vi "Beam Profiler.vi"(7 "Image Ref":T1) -> ()   [LabVIEW 2016]
uses:
  <vilib>/Utility/miscctls.llb/LVPointTypeDef.ctl
  <vilib>/vision/NI_Vision_Development_Module.lvlib
  <vilib>/vision/Image Controls.llb/IMAQ Image.ctl
panel:
  out "Y FWHM (px)":dbl=1.0
  out "X FWHM (px)":dbl=1.0
  out "Y FWHM (mm)":dbl=1.0
  out "X FWHM (mm)":dbl=1.0
  in  "Camera Pixel Size (µm)":dbl=1.0
  in  "Fitting":bool
  out "Fit":dbl[][](graph)
  out "Image":u16[][](graph)
  in  "Update Rate (ms)":i32=50
  in  "Binning (pixels)":i32=10 min=1 step=1
  in  "Done":bool
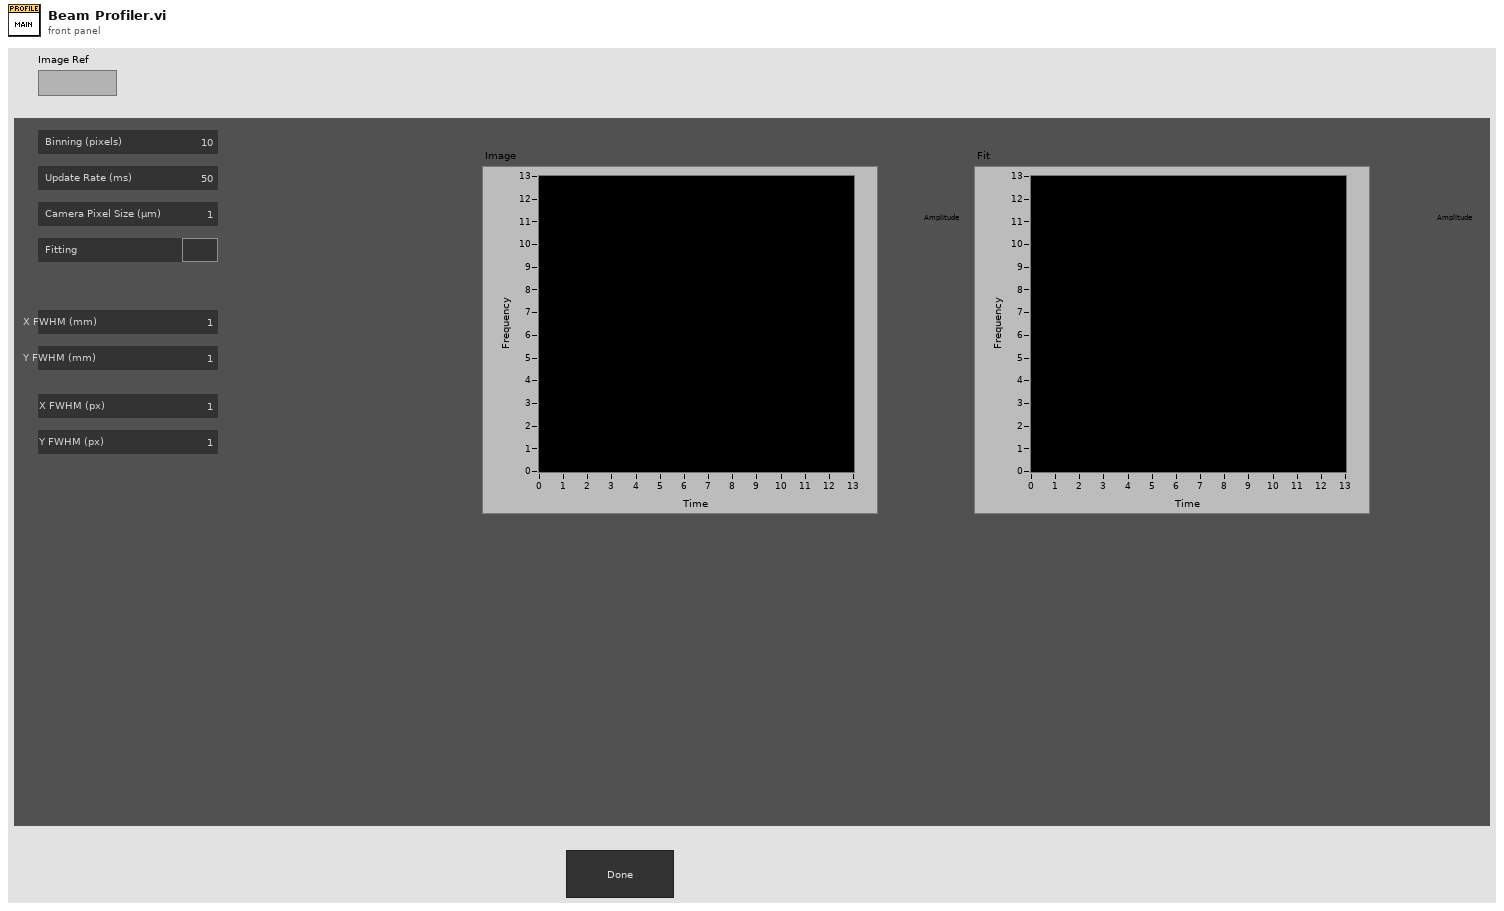
[diagram p1: front panel]
types:
  T1 = typedef "IMAQ Image.ctl" = refnum<image>
  T2 = typedef "Image Type" = u32
  T3 = enum16{"Always On", "Always Off", "Off While Running"}
  T4 = typedef "LVPointTypeDef.ctl" = cluster{"Horizontal":i16, "Vertical":i16}
  T5 = typedef "2D Gaussian - Best Fit Parameters.ctl" = cluster{"Amplitude":dbl, "X Position":dbl, "Y Position":dbl, "X Width":dbl, "Y Width":dbl, "Offset":dbl}
  T6 = typedef "LVRectTypeDef.ctl" = cluster{"Left":i16, "Top":i16, "Right":i16, "Bottom":i16}
  T7 = typedef "LVBoundsTypeDef.ctl" = cluster{"Width":u32, "Height":u32}
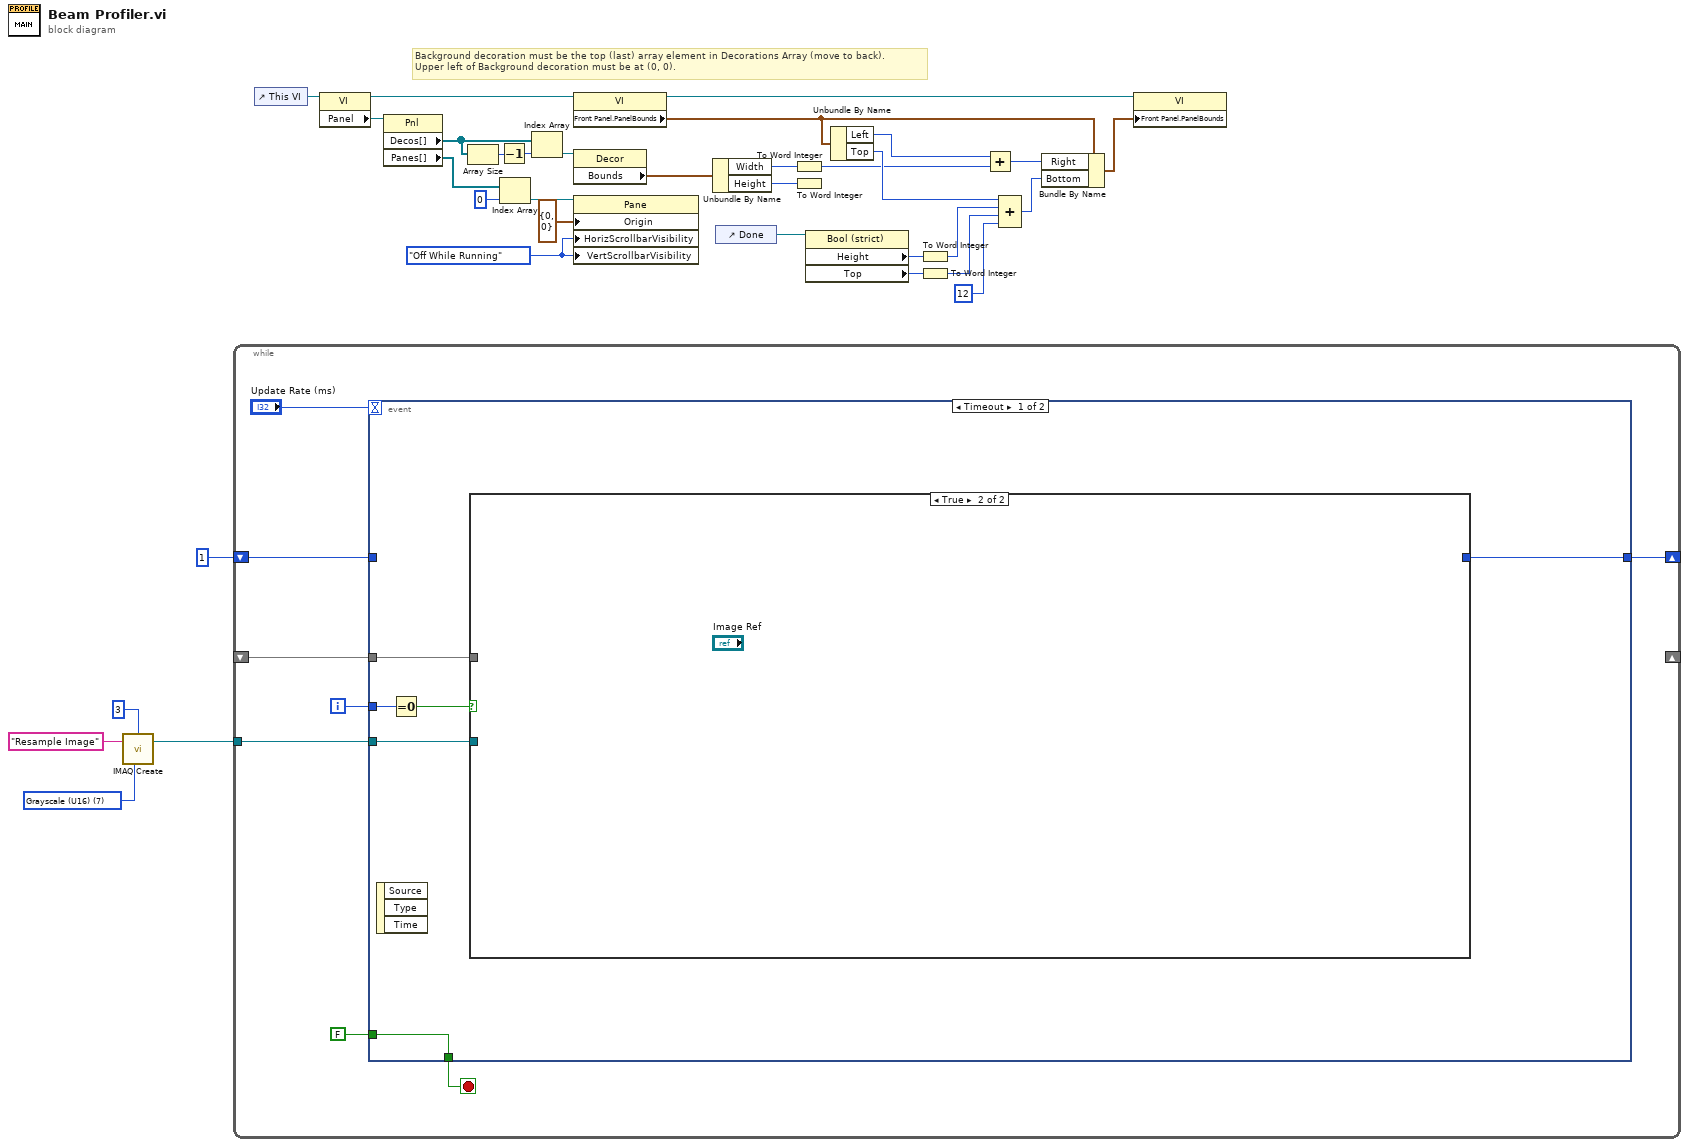
[diagram p0: block diagram]
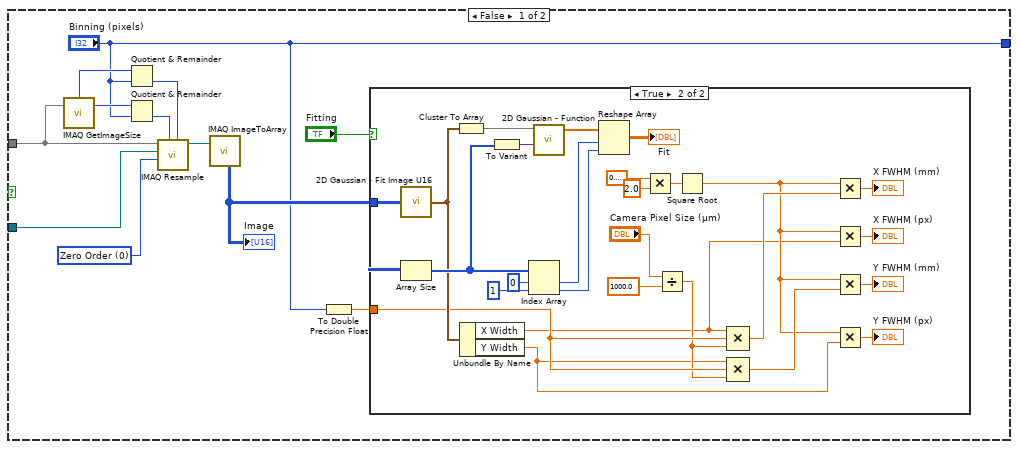
[diagram p2: hidden frame]
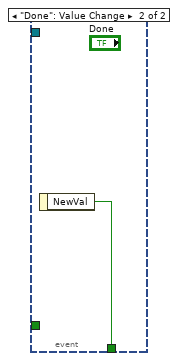
[diagram p4: hidden frame]
diagram:
  w5 = T2 7 items=["Grayscale (U8)", "Grayscale (I16)", "Grayscale (SGL)", "Complex (CSG)", "RGB (U32)", "HSL (U32)", "RGB (U64)", "Grayscale (U16)"] ("Image Type")
  w17 = T3."Off While Running" ("Vertical Scrollbar Visibility")
  # "Background decoration must be the top (last) array element in Decorations Array (move to back).\nUpper left of Background decoration must be at (0, 0)."
  n1 = call "IMAQ Create"("Border Size"=3, "Image Name"="Resample Image", "Image Type"=w5) -> ("New Image"=w2:T1)  [unwired: 2 in, 1 out]
  n2 = while {
    tunnel: w2 -> [w38]
    shift-right: _ -> [_]
    shift-left: _ -> [w39]
    shift-right: [w36] -> _
    shift-left: 1 ("Binning (pixels)") -> [w35]
    i -> [w37]
    stop <- w41 stop-if-true
    n3 = event shown="[0] Timeout" {
      selector: _ -> [_ _]
      dyn-events: _ -> [_ _]
      timeout: "Update Rate (ms)" -> [_ _]
      tunnel: [w48 w88] -> w41
      tunnel: FALSE -> [w48 _]
      tunnel: w39 -> [w46 _]
      tunnel: w38 -> [w47 _]
      tunnel: w37 -> [w45 _]
      tunnel: [w43 _] -> w36
      tunnel: w35 -> [_ _]
      event Timeout {
        n4 = event-data() -> ()  [unwired: 1 in, 3 out]
        n5 = Equal To 0?(x=w45) -> (x = 0?=w44:bool)
        n6 = case shown="True" w44 {
          tunnel: w47 -> [w60 _]
          tunnel: w46 -> [w57 _]
          tunnel: ["Binning (pixels)" _] -> w43
          frame False {
            w59 = u32 0 items=["Zero Order", "Bi-Linear", "Quadratic", "Cubic Spline"] ("Interpolation Type")
            n7 = call "IMAQ GetImageSize"("Image"=w57) -> ("Y Resolution"=w55:i32, "X Resolution"=w56:i32)  [unwired: 3 in, 1 out]
            n8 = Quotient & Remainder(x=w56, y="Binning (pixels)") -> (floor(x/y)=w54:i32)  [unwired: 1 out]
            n9 = Quotient & Remainder(x=w55, y="Binning (pixels)") -> (floor(x/y)=w53:i32)  [unwired: 1 out]
            n10 = call "IMAQ Resample"("X Resolution"=w54, "Y Resolution"=w53, "Interpolation Type"=w59, "Image Dst"=w60, "Image Src"=w57) -> ("Image Dst Out"=w58:T1)  [unwired: 5 in, 1 out]
            n11 = call "IMAQ ImageToArray"("Image"=w58) -> ("Image Pixels (U16)"=w52:u16[][])  [unwired: 3 in, 4 out]
            "Image" <- w52
            n12 = To Double Precision Float(number="Binning (pixels)") -> (double precision float=w50:dbl)
            n13 = case shown="True" "Fitting" {
              tunnel: w52 -> [_ w84]
              tunnel: w50 -> [_ w76]
              frame False {
              }
              frame True {
                n14 = call "2D Gaussian - Fit Image U16.vi"("Image In (U16)"=w84) -> ("Best Fit Params"=w77:T5)  [unwired: 13 in, 1 out]
                n15 = Array Size(array=w84) -> (size(s)=w78:i32[])
                n16 = Cluster To Array(cluster=w77) -> (array=w87:dbl[])
                n17 = Unbundle By Name(w77) -> ("X Width"=w67:dbl, "Y Width"=w66:dbl)
                n18 = To Variant(anything=w78) -> (Variant=w79:variant)
                n19 = Index Array(array=w78, index #1=0 ("index"), index #2=1 ("index")) -> (element #1=w81:i32, element #2=w80:i32)
                n20 = call "2D Gaussian - Function.vi"("data"=w79, "a"=w87) -> ("f(X,a)"=w86:dbl[])  [unwired: 2 in, 2 out]
                n21 = Reshape Array(w86, w81, w80) -> (→"Fit":dbl[][])
                n22 = Multiply(x=0.6931471805599453, y=2.0) -> (x*y=w71:dbl)
                n23 = Divide(x="Camera Pixel Size (µm)", y=1000.0) -> (x/y=w74:dbl)
                n24 = Square Root(x=w71) -> (sqrt(x)=w68:dbl)
                n25 = Compound Arithmetic op=MULTIPLY(w67, w76, w74) -> (w69:dbl)
                n26 = Compound Arithmetic op=MULTIPLY(w66, w76, w74) -> (w70:dbl)
                n27 = Multiply(x=w68, y=w69) -> (x*y=→"X FWHM (mm)":dbl)
                n28 = Multiply(x=w68, y=w67) -> (x*y=→"X FWHM (px)":dbl)
                n29 = Multiply(x=w68, y=w70) -> (x*y=→"Y FWHM (mm)":dbl)
                n30 = Multiply(x=w68, y=w66) -> (x*y=→"Y FWHM (px)":dbl)
              }
            }
          }
          frame True {
          }
        }
      }
      event "Done": Value Change {
        n31 = event-data() -> ("NewVal"=w88:bool)  [unwired: 1 in]
      }
    }
  }
  n32 = control-ref of="This VI"() -> (w9:refnum<vi>)
  n33 = property class="VI"(reference=w9) -> (reference out=w18:refnum<vi>, "Panel"=w10:refnum<vi>)  [unwired: 1 in, 1 out]
  n34 = property class="Pnl"(reference=w10) -> ("Decos[]"=w8:refnum<vi>[], "Panes[]"=w14:refnum<vi>[])  [unwired: 1 in, 2 out]
  n35 = Array Size(array=w8) -> (size(s)=w6:i32)
  n36 = Decrement(x=w6) -> (x-1=w7:i32)
  n37 = Index Array(array=w14, index=0) -> (element=w13:refnum<vi>)
  n38 = Index Array(array=w8, index=w7) -> (element=w16:refnum<vi>)
  n39 = property class="VI"(reference=w18) -> (reference out=w20:refnum<vi>, "Front Panel.PanelBounds"=w21:T6)  [unwired: 1 in, 1 out]
  n40 = property class="Decor"(reference=w16) -> ("Bounds"=w19:T7)  [unwired: 1 in, 2 out]
  n41 = property class="Pane"(reference=w13, "Origin"=T4 {"Horizontal"=0, "Vertical"=0}, "HorizScrollbarVisibility"=w17, "VertScrollbarVisibility"=w17) -> ()  [unwired: 1 in, 2 out]
  n42 = Unbundle By Name(w19) -> ("Width"=w24:u32, "Height"=w27:u32)
  n43 = control-ref of="Done"() -> (w11:refnum<vi>)
  n44 = To Word Integer(number=w24) -> (16bit integer=w26:i16)
  n45 = To Word Integer(number=w27) -> ()  [unwired: 1 out]
  n46 = property class="Bool (strict)"(reference=w11) -> ("Height"=w29:u32, "Top"=w30:i32)  [unwired: 1 in, 2 out]
  n47 = Unbundle By Name(w21) -> ("Left"=w23:i16, "Top"=w34:i16)
  n48 = To Word Integer(number=w29) -> (16bit integer=w32:i16)
  n49 = To Word Integer(number=w30) -> (16bit integer=w33:i16)
  n50 = Add(x=w23, y=w26) -> (x+y=w25:i16)
  n51 = Compound Arithmetic op=ADD(w34, w32, w33, i16 12 ("y")) -> (w28:i16)
  n52 = Bundle By Name(cluster=w21, "Right"=w25, "Bottom"=w28) -> (w22:T6)
  n53 = property class="VI"(reference=w20, "Front Panel.PanelBounds"=w22) -> ()  [unwired: 1 in, 2 out]
